vi "SoftFrontPanel.vi"(8 "error in (no error)":errorcluster, 11 "DMM Instrument":refnum<class "DMM Instrument.lvclass">) -> (0 "error out":errorcluster, 3 "DMM Instrument out":refnum<class "DMM Instrument.lvclass">)   [LabVIEW 2025, in "DMM.lvlib" / "DMM Instrument.lvclass"]
doc: "Copyright 2017 National Instruments Corporation\n\nLicensed under the Apache License, Version 2.0 (the \"License\"); you may not use this file except in compliance with the License. You may obtain a copy of the License at http://www.apache.org/licenses/LICENSE-2.0\nUnless required by applicable law or agreed to in writing, software distributed under the License is distributed on an \"AS IS\" BASIS, WITHOUT WARRANTIES OR CONDITIONS OF ANY KIND, either express or implied. See the License for the specific language governing permissions and limitations under the License."
uses:
  DMM Instrument.lvclass
  DMM Instrument.lvclass/DMM Instrument.ctl
  DMM configuration/DMM configuration.lvclass
  Users/Public/Documents/Sandia National Labs/TSS Plugin/Abstract Engine.lvlibp/Instrument configuration/Read Instrument Setting.vi
  Users/Public/Documents/Sandia National Labs/TSS Plugin/CEF.lvlibp/Node/ReadChildren.vi
  Users/Public/Documents/Sandia National Labs/TSS Plugin/CEF.lvlibp/Node/CEF_Node.lvclass
  <vilib>/Analysis/baseanly.llb/Mean (DBL).vi
  <vilib>/Analysis/NI_AALBase.lvlib
panel:
  in  "Channels":enum32{"Ch0", "Ch1", "Ch2", "Ch3"}(radio)
  out "Instrument":cluster{"Chname":string, "Voltage":dbl}={"Chname"="Ch0", "Voltage"=0.0} {"Voltage" format="%#_4f"}
  out "Instrument":string caption="Instrument ::"
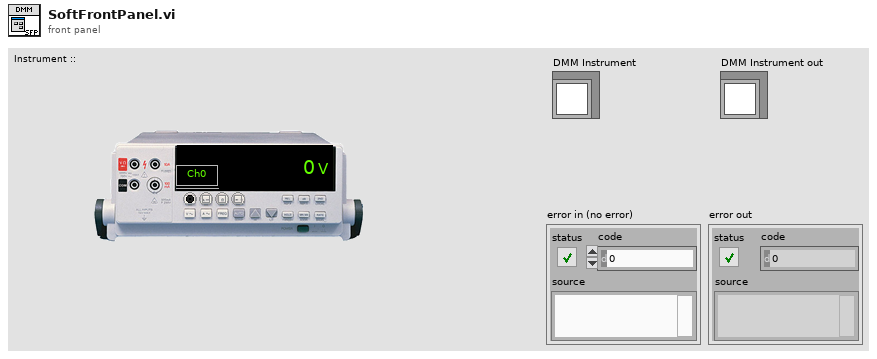
[diagram p1: front panel]
types:
  T1 = enum32{"Invalid", "Default", "Floating", "Floating/Auto-Hide", "Modal"}
  T2 = typedef "Abstract Engine.lvlibp/Instrument configuration.lvclass/Default Instrument.ctl" = cluster{"Type":string, "Address":string, "SW Alias":string, "Description":string, "Enabled":bool}
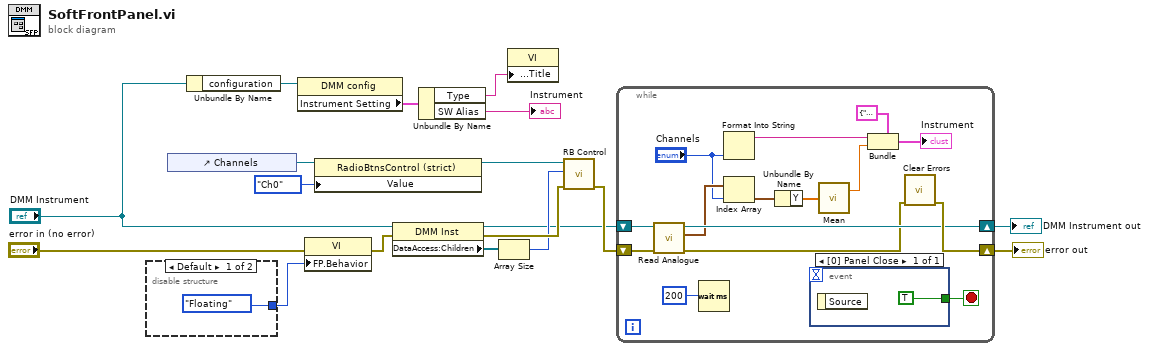
[diagram p0: block diagram]
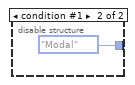
[diagram p2: hidden frame]
diagram:
  n1 = disable-structure shown="Default" {
    disable-tunnel: [T1."Floating" ("Front Panel Window:Behavior") T1."Modal" ("Front Panel Window:Behavior")] -> w16
    frame condition #0 (active) {
    }
    frame condition #1 {
    }
  }
  n2 = control-ref of="Channels"() -> (w7:refnum<vi>)
  n3 = Unbundle By Name("DMM Instrument") -> ("configuration"=w15:refnum<class "DMM configuration.lvclass">)
  n4 = property class="DMM config"(reference=w15) -> ("Instrument Setting"=w14:T2)  [unwired: 1 in, 2 out]
  n5 = property class="VI"(error in="error in (no error)", "FP.Behavior"=w16) -> (error out=w12:errorcluster)  [unwired: 1 in, 1 out]
  n6 = property class="RadioBtnsControl (strict)"(reference=w7, "Value"=enum32{"Ch0", "Ch1", "Ch2", "Ch3"}."Ch0") -> (reference out=w4:refnum<vi>)  [unwired: 1 in, 1 out]
  n7 = property class="DMM Inst"(reference="DMM Instrument", error in=w12) -> (reference out=w5:refnum<class "DMM Instrument.lvclass">, error out=w10:errorcluster, "DataAccess:Children"=w11:refnum<data-value>[])
  n8 = Unbundle By Name(w14) -> ("Type"=w13:string, "SW Alias"=→"Instrument":string)
  n9 = Array Size(array=w11) -> (size(s)=w8:i32)
  n10 = property class="VI"("Front Panel.Title"=w13) -> ()  [unwired: 2 in, 2 out]
  n11 = call "RB Control.vi"("error in"=w10, "Channels"=w8, "Radio Ref"=w4) -> ("error out"=w9:errorcluster)  [unwired: 8 in]
  n12 = while {
    shift-right: [w34] -> w18
    shift-left: w9 -> [w35]
    shift-right: [w32] -> w1
    shift-left: w5 -> [w33]
    stop <- w21 stop-if-true
    n13 = call-dynamic "Read Analogue.vi"("error in (no error)"=w35, "Abstract DMM in"=w33) -> ("error out"=w28:errorcluster, "Waveforms"=w30:waveform(dbl)[], "Abstract DMM out"=w32:refnum<class "DMM Instrument.lvclass">)  [unwired: 7 in]
    n14 = Wait (ms)(milliseconds to wait=u32 200) -> ()  [unwired: 1 out]
    n15 = Format Into String("Channels") -> (resulting string=w27:string)  [unwired: 3 in, 1 out]
    n16 = Index Array(array=w30, index="Channels") -> (element=w25:waveform(dbl))
    n17 = Unbundle By Name(w25) -> ("Y"=w24:dbl[])
    n18 = event shown="[0] Panel Close" {
      selector: _ -> [_]
      dyn-events: _ -> [_]
      timeout: _ -> [_]
      tunnel: [TRUE] -> w21
      event Panel Close {
        n19 = event-data() -> ()  [unwired: 1 in, 1 out]
      }
    }
    n20 = call-poly <vilib>:"Mean.vi"("X"=w24) -> ("mean"=w23:dbl)  [unwired: 1 out]
    n21 = Bundle(cluster=cluster{string, "mean":dbl} {"", "mean"=nan}, w27, "mean"=w23) -> (→"Instrument":cluster{string, "mean":dbl})
    n22 = call <vilib>:"Clear Errors.vi"("error in (no error)"=w28) -> ("error out"=w34:errorcluster)  [unwired: 5 in, 1 out]
  }
  "error out" <- w18
  "DMM Instrument out" <- w1
